vi "LinearSystemSim_GetOutput.vi"(11 "LinearSysemSim":T2) -> (3 "Output":T1)   [LabVIEW 2019, in "Trajectory_Library.lvlib"]
doc: "Returns the current output of the plant.\n \nInputs:\n - LinearSystemSim -- Data cluster\n\nOutputs:\n - Output -- The current output matrix of the plant."
uses:
  Trajectory_Library.lvlib
  TypeDef/LINEAR_SYSTEM.ctl
  <vilib>/Analysis/Matrix/Datatypes/RealMatrix.ctl
  <vilib>/Analysis/Matrix/NI_Matrix.lvlib
  TypeDef/LINEAR_SYSTEM_SIM.ctl
panel:
  # "<States, 1>"
  # "<Outputs, 1>"
  # "<Inputs, 1>"
  # "<Outputs, 1>"
  # "<States,States>"
  # "<States,Inputs>"
  # "<Outputs,States>"
  # "<Outputs,Inputs>"
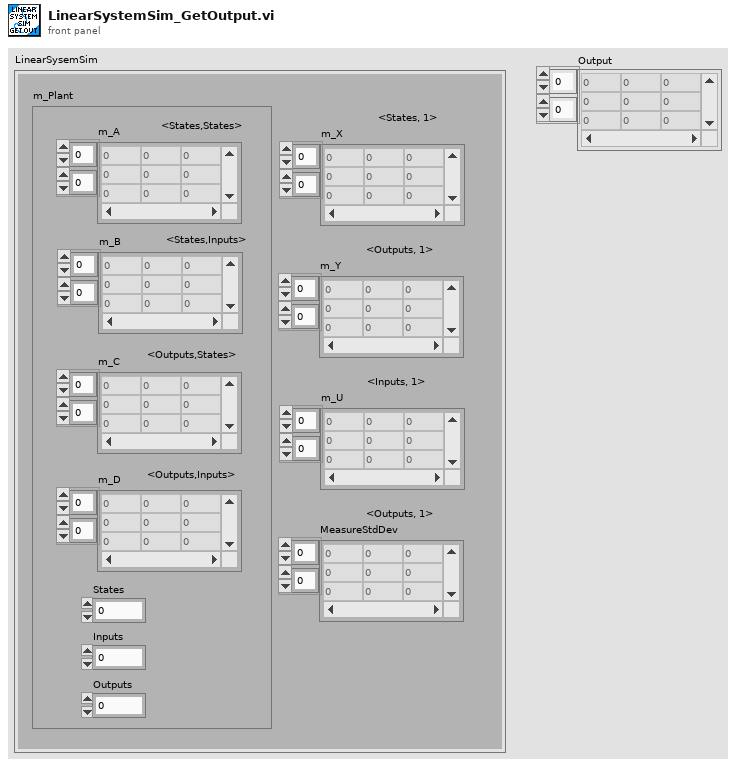
[diagram p1: front panel]
types:
  T1 = typedef "NI_Matrix.lvlib/RealMatrix.ctl" = dbl[][]
  T2 = typedef "Trajectory_Library.lvlib/LINEAR_SYSTEM_SIM.ctl" = cluster{"m_Plant":T3, "m_X":T1, "m_Y":T1, "m_U":T1, "MeasureStdDev":T1}
  T3 = typedef "Trajectory_Library.lvlib/LINEAR_SYSTEM.ctl" = cluster{"m_A":T1, "m_B":T1, "m_C":T1, "m_D":T1, "States":i32, "Inputs":i32, "Outputs":i32}
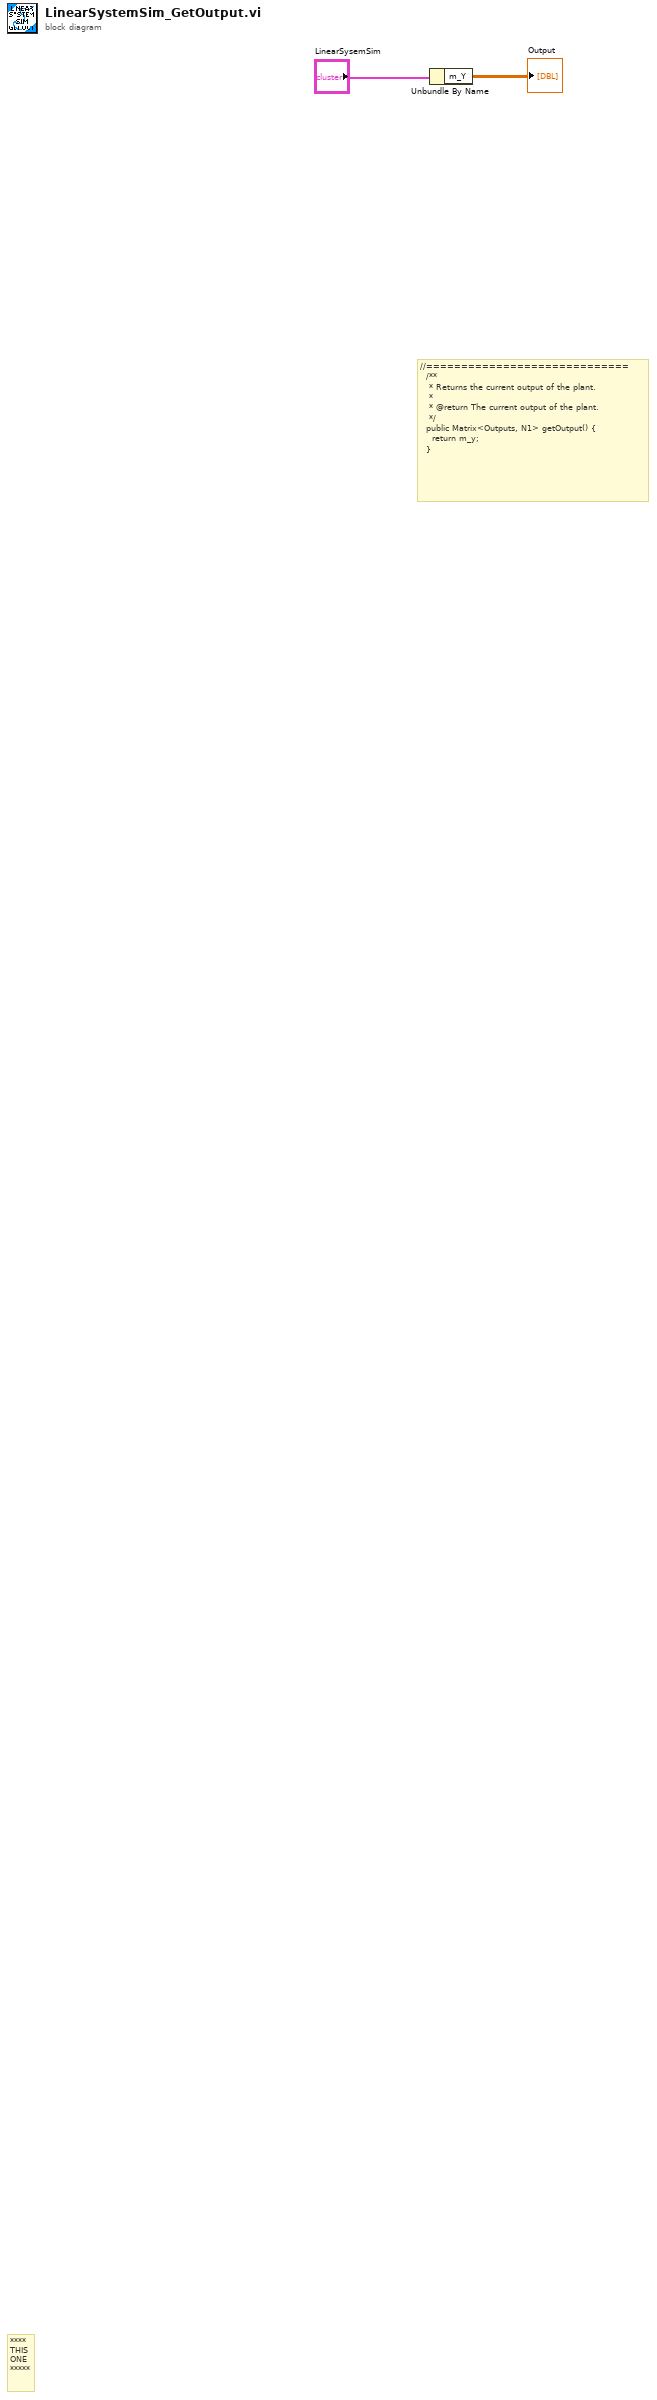
[diagram p0: block diagram]
diagram:
  # "//=============================\n  /**\n   * Returns the current output of the plant.\n   *\n   * @return The current output of the plant.\n   */\n  public Matrix<Outputs, N1> getOutput() {\n    return m_y;\n  }"
  # "****\nTHIS\nONE\n*****"
  n1 = Unbundle By Name("LinearSysemSim") -> ("m_Y"=→"Output":T1)
